vi "AC Table save for TDMS.vi"(8 "error in":errorcluster, 9 "AC Table Tag":string[](array[string]), 10 "Set Condition":T1={"+/- Point"=2000, "Cut Region"=500, "BL Selection"=enum."Div Value Mode BL", "STD Selection"=enum."DivSTD Mode STD", "D Th std xn"=1.0, "U Th std xn"=6.0, "MAX D time (ms)"=10.0, "LL BR (n)"=0, "LL BR T length (ms)"=0.0, "LL Retention (ms)"=0.0, "Read Region Point"=10000, "Filter Selection"=enum."Mean", "STD smooth Point"=10, "MAX E_S time (ms)"=10.0}, 11 "TDMSファイル in":refnum<k34>) -> (0 "error out":errorcluster, 3 "TDMSファイル out":refnum<k34>)   [LabVIEW 2018]
panel:
  out "AC Table Data":string[](array[string])
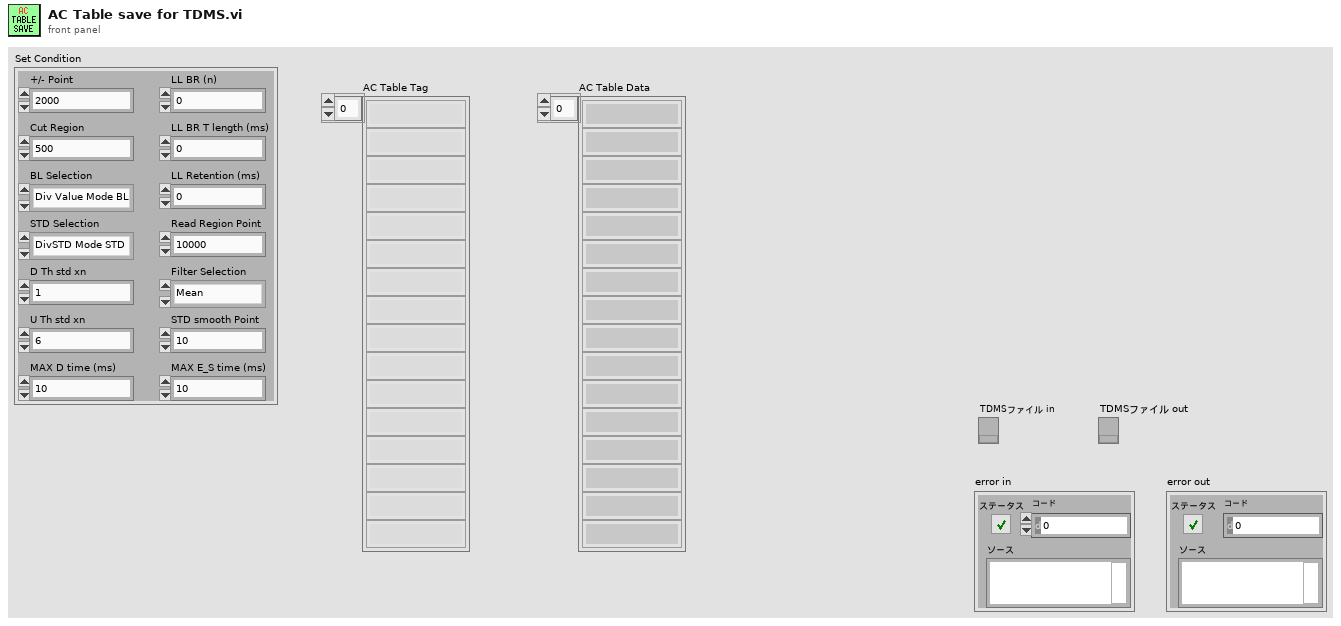
[diagram p1: front panel]
types:
  T1 = cluster{"+/- Point":i32, "Cut Region":i32, "BL Selection":enum16{"All Value Mode BL", "Div Value Mode BL", "Div Mean Mean BL", "Min Peak Value BL"}, "STD Selection":enum16{"All Value STD", "Div STD Mean STD", "DivSTD Mode STD"}, "D Th std xn":dbl, "U Th std xn":dbl, "MAX D time (ms)":dbl, "LL BR (n)":i32, "LL BR T length (ms)":dbl, "LL Retention (ms)":dbl, "Read Region Point":i32, "Filter Selection":enum16{"Mean", "Smooth"}, "STD smooth Point":i32, "MAX E_S time (ms)":dbl}
  T2 = enum16{"All Value Mode BL", "Div Value Mode BL", "Div Mean Mean BL", "Min Peak Value BL"}
  T3 = enum16{"All Value STD", "Div STD Mean STD", "DivSTD Mode STD"}
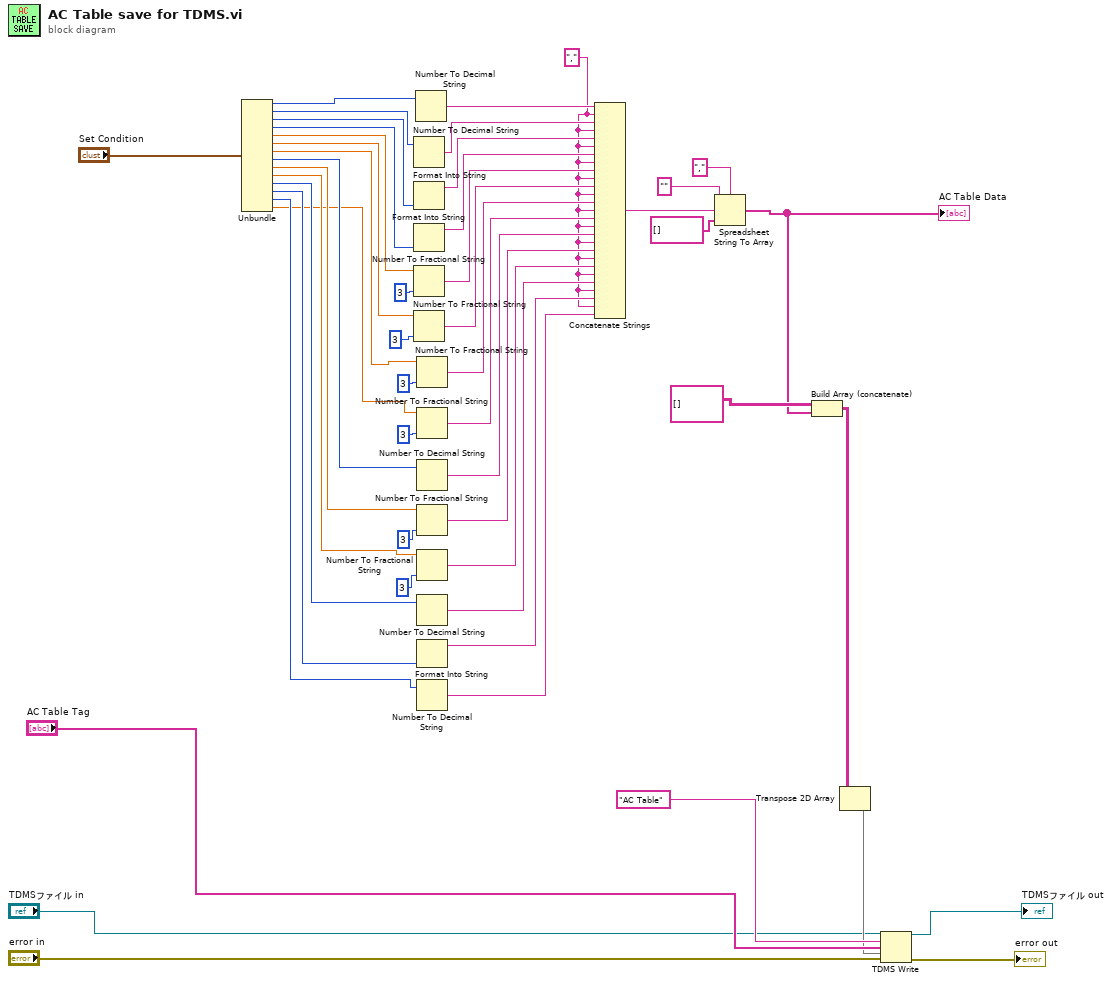
[diagram p0: block diagram]
diagram:
  w8 = "," ("デリミタ（タブ）")
  n1 = Unbundle("Set Condition") -> ("+/- Point"=w49:i32, "Cut Region"=w48:i32, "BL Selection"=w47:T2, "STD Selection"=w46:T3, "D Th std xn"=w45:dbl, "U Th std xn"=w42:dbl, "MAX D time (ms)"=w31:dbl, "LL BR (n)"=w41:i32, "LL BR T length (ms)"=w38:dbl, "LL Retention (ms)"=w37:dbl, "Read Region Point"=w36:i32, "Filter Selection"=w35:enum16{"Mean", "Smooth"}, "STD smooth Point"=w34:i32, "MAX E_S time (ms)"=w30:dbl)
  n2 = Number To Decimal String(number=w48) -> (decimal integer string=w28:string)  [unwired: 1 in]
  n3 = Format Into String(w47) -> (resulting string=w27:string)  [unwired: 3 in, 1 out]
  n4 = Format Into String(w46) -> (resulting string=w26:string)  [unwired: 3 in, 1 out]
  n5 = Number To Fractional String(number=w45, precision (6)=i16 3 ("精度（6）")) -> (F-format string=w25:string)  [unwired: 2 in]
  n6 = Number To Fractional String(number=w42, precision (6)=i16 3 ("精度（6）")) -> (F-format string=w24:string)  [unwired: 2 in]
  n7 = Number To Decimal String(number=w49) -> (decimal integer string=w29:string)  [unwired: 1 in]
  n8 = Number To Fractional String(number=w31, precision (6)=i16 3 ("精度（6）")) -> (F-format string=w23:string)  [unwired: 2 in]
  n9 = Number To Fractional String(number=w30, precision (6)=i16 3 ("精度（6）")) -> (F-format string=w22:string)  [unwired: 2 in]
  n10 = Number To Decimal String(number=w41) -> (decimal integer string=w21:string)  [unwired: 1 in]
  n11 = Number To Fractional String(number=w38, precision (6)=i16 3 ("精度（6）")) -> (F-format string=w20:string)  [unwired: 2 in]
  n12 = Number To Fractional String(number=w37, precision (6)=i16 3 ("精度（6）")) -> (F-format string=w19:string)  [unwired: 2 in]
  n13 = Number To Decimal String(number=w36) -> (decimal integer string=w18:string)  [unwired: 1 in]
  n14 = Format Into String(w35) -> (resulting string=w17:string)  [unwired: 3 in, 1 out]
  n15 = Number To Decimal String(number=w34) -> (decimal integer string=w16:string)  [unwired: 1 in]
  n16 = Concatenate Strings(w29, w8, w28, w8, w27, w8, w26, w8, w25, w8, w24, w8, w23, w8, w22, w8, w21, w8, w20, w8, w19, w8, w18, w8, w17, w8, w16) -> (w12:string)
  n17 = Spreadsheet String To Array(delimiter (Tab)="," ("デリミタ（タブ）"), format string="" ("形式文字列"), spreadsheet string=w12, array type (2D Dbl)=string[] [] ("行ヘッダ文字列[]")) -> (array=w6:string[])
  "AC Table Data" <- w6
  n18 = Build Array (concatenate)(string[][] [] ("Table"), w6) -> (w5:string[][])
  n19 = Transpose 2D Array(2D array=w5) -> (transposed array=w3:string[][])
  n20 = TDMS Write(0:"TDMSファイル in", 5:"AC Table" ("Group name"), 7:"AC Table Tag", 9:w3, 11:"error in") -> (4:→"TDMSファイル out":refnum<k34>, 15:→"error out":errorcluster)  [unwired: 1 in, 2 out]
